vi "Run.vi"(8 "error in (no error)":errorcluster, 10 "UI Refs":T1, 11 "4way Leakage":refnum<class "Leakage.lvclass">) -> (0 "error out":errorcluster, 3 "4way Leakage out":refnum<class "Leakage.lvclass">)   [LabVIEW 2025, in "Flow Grind.lvlib" / "Leakage.lvclass"]
uses:
  Leakage.lvclass
  Leakage.lvclass/Leakage.ctl
  Users/Public/Documents/Sandia National Labs/TSS Plugin/Tests/XY Plotter.lvlibp/XY  Plotter/XY Plotter.lvclass
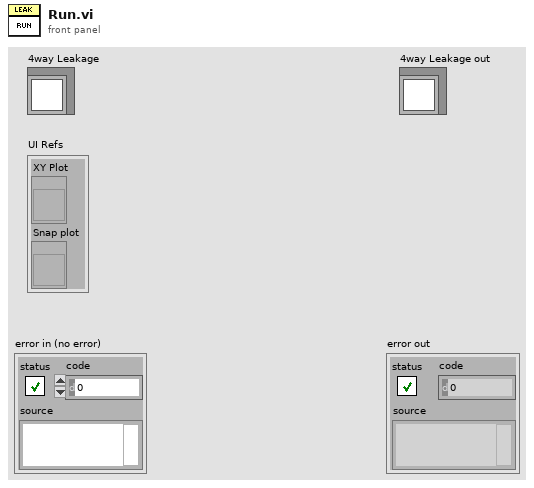
[diagram p1: front panel]
types:
  T1 = cluster{"XY Plot":refnum<vi>, "Snap plot":refnum<vi>}
  T2 = cluster{"Name":string, "Color":u32, "Style":u8, "Point Style":u8, "Name Visible":bool, "Allow Drag":bool, "Annotation Mode":u32, "Plot":i32, "Index":i32, "Position":cluster{"X":dbl, "Y":dbl}, "X Scale":u32, "Y Scale":u32, "Show Arrow":bool, "Lock Name":bool, "Plot Area":i32, "Label Offset":cluster{"X":dbl, "Y":dbl}}
  T3 = typedef "LVAnnotationListTypeDef.ctl" = cluster{"Name":string, "Color":u32, "Style":u8, "Point Style":u8, "Name Visible":bool, "Allow Drag":bool, "Annotation Mode":u32, "Plot":i32, "Index":i32, "Position":cluster{"X":dbl, "Y":dbl}, "X Scale":u32, "Y Scale":u32, "Show Arrow":bool, "Lock Name":bool, "Plot Area":i32, "Label Offset":cluster{"X":dbl, "Y":dbl}}[]
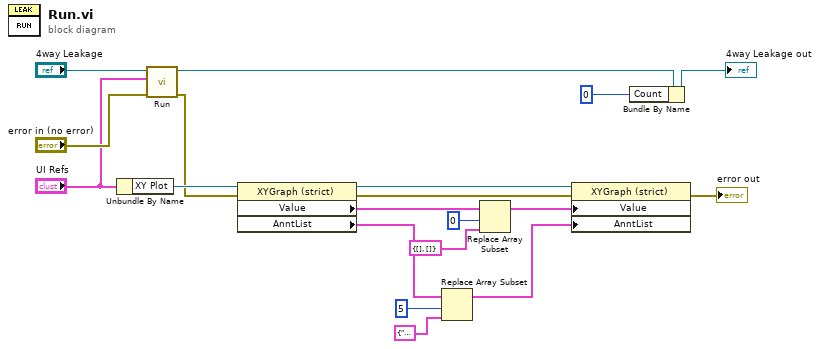
[diagram p0: block diagram]
diagram:
  n1 = Unbundle By Name("UI Refs") -> ("XY Plot"=w12:refnum<vi>)
  n2 = call-parent "Run.vi"("error in (no error)"="error in (no error)", "UI Refs"="UI Refs", "XY Plotter"="4way Leakage") -> ("error out"=w11:errorcluster, "XY Plotter out"=w16:refnum<class "Leakage.lvclass">)  [unwired: 7 in]
  n3 = property class="XYGraph (strict)"(reference=w12) -> (reference out=w9:refnum<vi>, "Value"=w8:cluster{"Wavenumber":dbl[], "Data":dbl[]}[], "AnntList"=w2:T3)  [unwired: 1 in, 1 out]
  n4 = Replace Array Subset(array=w2, new element=T2 {"Name"="", "Color"=0, "Style"=0, "Point Style"=0, "Name Visible"=FALSE, "Allow Drag"=FALSE, "Annotation Mode"=0, "Plot"=0, "Index"=0, "Position"={"X"=0.0, "Y"=0.0}, "X Scale"=0, "Y Scale"=0, "Show Arrow"=FALSE, "Lock Name"=FALSE, "Plot Area"=0, "Label Offset"={"X"=0.0, "Y"=0.0}} ("new element/subarray"), index=5) -> (w1:T3)
  n5 = Replace Array Subset(array=w8, new element=cluster{"Wavenumber":dbl[], "Data":dbl[]} {"Wavenumber"=[], "Data"=[]} ("Spectrum"), index=0) -> (w7:cluster{"Wavenumber":dbl[], "Data":dbl[]}[])
  n6 = property class="XYGraph (strict)"(reference=w9, error in=w11, "Value"=w7, "AnntList"=w1) -> (error out=→"error out":errorcluster)  [unwired: 1 out]
  n7 = Bundle By Name(cluster=w16, "Count"=0) -> (→"4way Leakage out":refnum<class "Leakage.lvclass">)
